vi "case struture.vi"() -> ()   [LabVIEW 2021]
panel:
  out "OUTPUT":dbl
  in  "CONTROL":i32
  in  "B":dbl
  in  "A":dbl
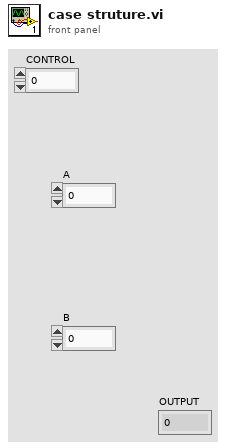
[diagram p1: front panel]
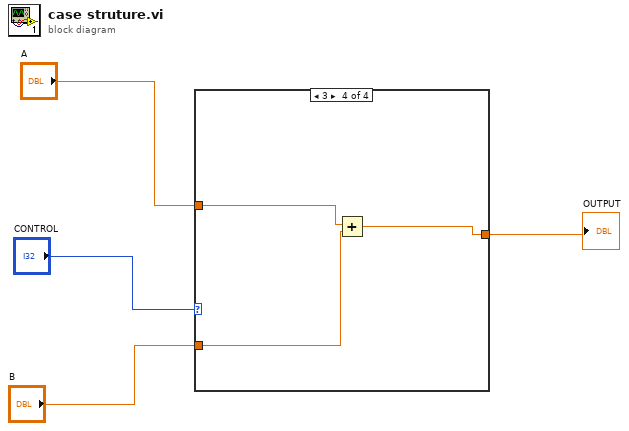
[diagram p0: block diagram]
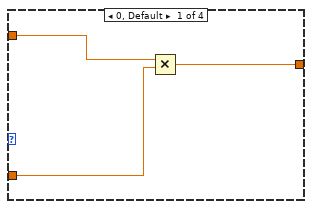
[diagram p2: hidden frame]
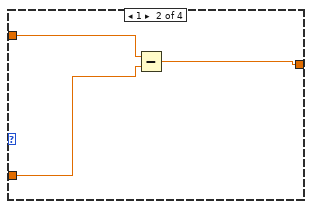
[diagram p3: hidden frame]
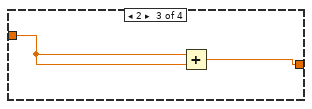
[diagram p4: hidden frame]
diagram:
  n1 = case shown="3" "CONTROL" {
    tunnel: "A" -> [w6 w10 w11 w15]
    tunnel: "B" -> [w7 w9 _ w14]
    tunnel: [w5 w8 w12 w13] -> w1
    frame 0, Default {
      n2 = Multiply(x=w6, y=w7) -> (x*y=w5:dbl)
    }
    frame 1 {
      n3 = Subtract(x=w10, y=w9) -> (x-y=w8:dbl)
    }
    frame 2 {
      n4 = Add(x=w11, y=w11) -> (x+y=w12:dbl)
    }
    frame 3 {
      n5 = Add(x=w15, y=w14) -> (x+y=w13:dbl)
    }
  }
  "OUTPUT" <- w1
